vi "Load Patterns to Sessions.vi"(8 "error in":errorcluster, 10 "pattern file paths":string[](array[string]), 11 "sequence context":refnum<k7>) -> (0 "error out":errorcluster)   [LabVIEW 2021, in "NIDigitalSPI.lvlib"]
uses:
  NIDigitalSPI.lvlib
  <vilib>/Plug-In SDKs/Clients/Session Management V1/Session Reservation/Initialize and Close Session Behavior.ctl
  <vilib>/Plug-In SDKs/Clients/Session Management V1/Session Reservation/Session Reservation.lvclass
  <vilib>/Plug-In SDKs/Sessions/niDigital/NI Session Management niDigital.lvlib
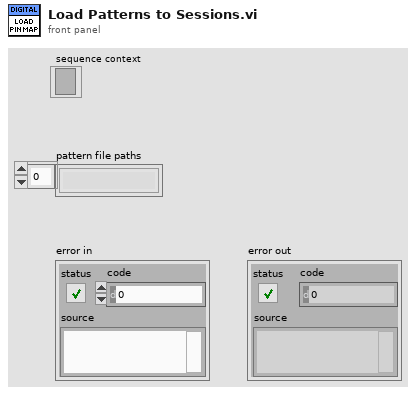
[diagram p1: front panel]
types:
  T1 = typedef "NI Session Management V1 Client.lvlib/Session Reservation.lvclass/Initialize and Close Session Behavior.ctl" = enum16{"Auto", "Initialize and Close", "Attach and Detach", "Initialize and Detach", "Attach and Close"}
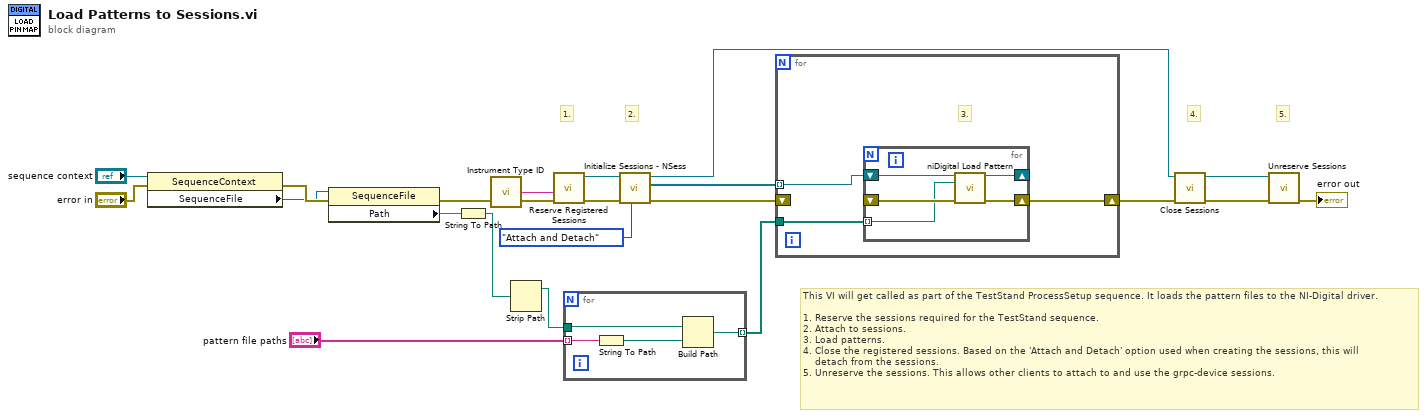
[diagram p0: block diagram]
diagram:
  # "5."
  # "2."
  # "1."
  # "4."
  # "This VI will get called as part of the TestStand ProcessSetup sequence. It loads the pattern files to the NI-Digital driver.\n\n1. Reserve the sessions required for the TestStand sequence.\n2. Attach to sessions.\n3. Load patterns.\n4. Close the registered sessions. Based on the 'Attach and Detach' option used when creating the sessions, this will\n    detach from the sessions.\n5. Unreserve the sessions. This allows other clients to attach to and use the grpc-device sessions."
  n1 = property class="SequenceContext"(reference="sequence context", error in="error in") -> (error out=w21:errorcluster, "SequenceFile"=w20:refnum<k7>)  [unwired: 1 out]
  n2 = property class="SequenceFile"(reference=w20, error in=w21) -> (error out=w10:errorcluster, "Path"=w19:string)  [unwired: 1 out]
  n3 = String To Path(string=w19) -> (path=w16:path)
  n4 = call <vilib>:"Instrument Type ID.vi"() -> ("instrument type id"=w6:string)  [unwired: 5 in]
  n5 = Strip Path(path=w16) -> (stripped path=w14:path)  [unwired: 1 out]
  n6 = call <vilib>:"Reserve Registered Sessions.vi"("error in"=w10, "instrument type id"=w6) -> ("error out"=w12:errorcluster, "session reservation out"=w11:refnum<class "Session Reservation.lvclass">)  [unwired: 8 in]
  n7 = for {
    tunnel: "pattern file paths" -> [w25] mode=indexing
    tunnel: [w22] -> w13 mode=indexing
    tunnel: w14 -> [w24]
    n8 = String To Path(string=w25) -> (path=w23:path)
    n9 = Build Path(base path=w24, name or relative path=w23) -> (appended path=w22:path)
  }
  n10 = call <vilib>:"Initialize Sessions - NSess.vi"("initialize and close session behavior"=Initialize_and_Close_Session_Behavior."Attach and Detach", "error in"=w12, "session reservation in"=w11) -> ("error out"=w8:errorcluster, "sessions"=w9:refnum<k15>[], "session reservation out"=w3:refnum<class "Session Reservation.lvclass">)  [unwired: 5 in, 1 out]
  n11 = for {
    shift-right: [w26] -> w4
    shift-left: w8 -> [_]
    tunnel: w13 -> [w28]
    tunnel: w9 -> [w27] mode=indexing
    # "3."
    n12 = for {
      shift-right: [w33] -> w26
      shift-left: _ -> [w31]
      shift-right: [w32] -> _
      shift-left: w27 -> [w30]
      tunnel: w28 -> [w29] mode=indexing
      n13 = call <instrlib>:"niDigital Load Pattern.vi"("instrument handle"=w30, "pattern file"=w29, "error in"=w31) -> ("instrument handle out"=w32:refnum<k15>, "error out"=w33:errorcluster)  [unwired: 11 in]
    }
  }
  n14 = call <vilib>:"Close Sessions.vi"("error in"=w4, "session reservation in"=w3) -> ("error out"=w1:errorcluster, "session reservation out"=w2:refnum<class "Session Reservation.lvclass">)  [unwired: 8 in]
  n15 = call <vilib>:"Unreserve Sessions.vi"("error in"=w1, "session reservation in"=w2) -> ("error out"=→"error out":errorcluster)  [unwired: 9 in]
